vi "USBTC08OpenUnit.vi"(8 "error in (no error)":errorcluster) -> (0 "error out":errorcluster, 3 "Handle out":i16)   [LabVIEW 2010]
uses:
  usbtc08.dll
panel:
  out "Handle":i16
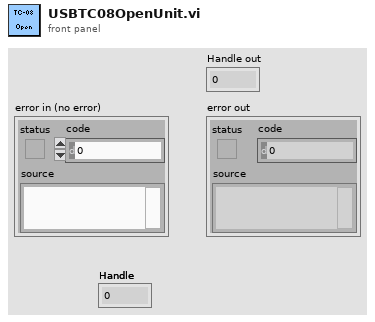
[diagram p1: front panel]
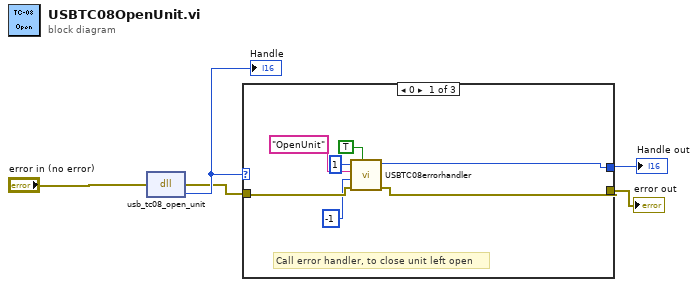
[diagram p0: block diagram]
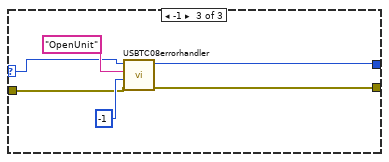
[diagram p3: hidden frame]
diagram:
  n1 = dll-call lib="usbtc08.dll" fn="usb_tc08_open_unit" label="OpenUnit"(error in="error in (no error)") -> (error out=w3:errorcluster, "Handle"=w5:i16)  [unwired: 2 in, 1 out]
  "Handle" <- w5
  n2 = case shown="0" w5 {
    selector: w5 -> [_ w14 w16]
    tunnel: [w6 w14 w15] -> w4
    tunnel: w3 -> [w12 w13 w18]
    tunnel: [w11 w13 w17] -> w1
    frame 0 {
      # "Call error handler, to close unit left open"
      n3 = call "USBTC08errorhandler.vi"("Close unit"=TRUE, "error in (no error)"=w12, "Return"=i16 -1, "API function"="OpenUnit", "Handle in"=i16 1) -> ("error out"=w11:errorcluster, "Handle out"=w6:i16)  [unwired: 5 in]
    }
    frame 1, Default {
      # "Any valid handle value >0"
    }
    frame -1 {
      n4 = call "USBTC08errorhandler.vi"("error in (no error)"=w18, "Return"=i16 -1, "API function"="OpenUnit", "Handle in"=w16) -> ("error out"=w17:errorcluster, "Handle out"=w15:i16)  [unwired: 6 in]
    }
  }
  "Handle out" <- w4
  "error out" <- w1
